vi "VIH - CHM Project - Create Project Files.vi"(8 "error in":errorcluster, 10 "HHP_Generation":T1={"HHP_Template"=enum."default", "HHP_Template_CustomPath"=path "", "HHP_Target"=enum."default", "HHP_Target_CustomPath"=path "", "HHP_CreateTOC"=TRUE, "HHP_CreateIDX"=TRUE, "HHP_DefaultTopic"=enum."auto", "HHP_DefaultTopic_CustomPath"=path "", "CHM_Filename"=path "", "HHP_AutoBuild"=FALSE, "CHM_AutoBuild"=FALSE}, 11 "Project Tree":T2) -> (0 "error out":errorcluster, 2 "Target HHP File":path, 3 "dup Project Tree":T2)   [LabVIEW 2014]
doc: "::: VI Helpeks :::\nCopyright (c) 2000-2026 Konstantin Shifershteyn. All rights reserved."
uses:
  _VIH Project Manager.llb/VIH Project Tree Typedef - Tree Refnum.ctl
  VIH - CHM Project - HHP Generation Params Cluster.ctl
panel:
  # "VI Helpeks\nCopyright (c) 2012-2026 Konstantin Shifershteyn"
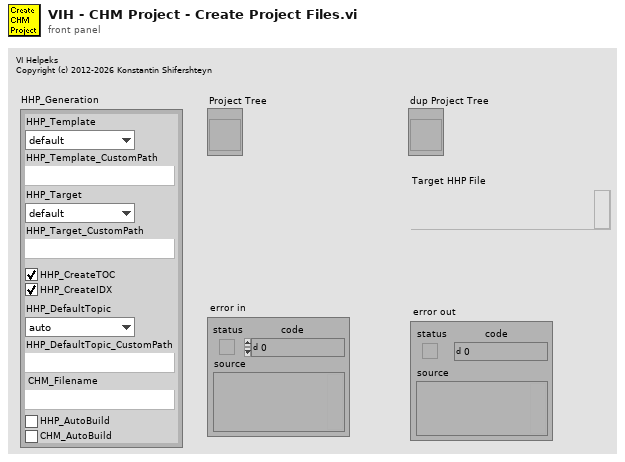
[diagram p1: front panel]
types:
  T1 = typedef "VIH - CHM Project - HHP Generation Params Cluster.ctl" = cluster{"HHP_Template":enum16{"default", "custom"}, "HHP_Template_CustomPath":path, "HHP_Target":enum16{"default", "custom"}, "HHP_Target_CustomPath":path, "HHP_CreateTOC":bool, "HHP_CreateIDX":bool, "HHP_DefaultTopic":enum16{"auto", "custom"}, "HHP_DefaultTopic_CustomPath":path, "CHM_Filename":path, "HHP_AutoBuild":bool, "CHM_AutoBuild":bool}
  T2 = typedef "VIH Project Tree Typedef - Tree Refnum.ctl" = refnum<vi>
  T3 = cluster{"TOC File":path, "IDX File":path, "HTML Files":path[], "Default Topic File":path, "Compiled File":path}
  T4 = typedef "VIH HelpGen Typedef - Palette - Item Type Enum.ctl" = enum32{"<Invalid>", "<unknown>", "VI", "Menu", "LV Func", "Express VI", "Poly VI", "CTL", "HTML"}
  T5 = cluster{"Types":T4[], "Src Paths":path[], "Dynamic":enum16{"Dyn", "Stat", "Both"}[], "HTML Paths":path[], "HTML Titles":string[]}
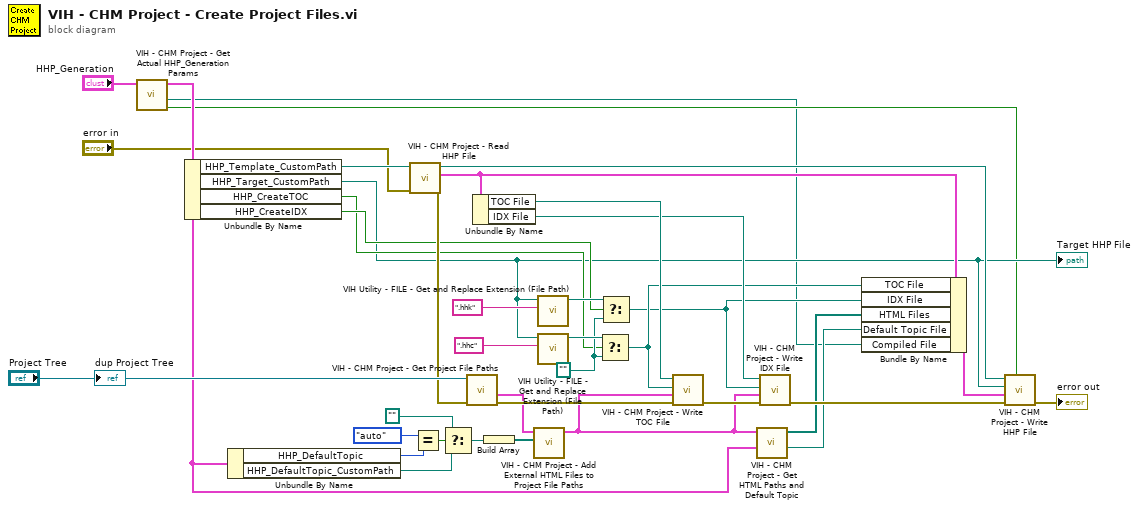
[diagram p0: block diagram]
diagram:
  w24 = path ""
  n1 = call "VIH - CHM Project - Get Actual HHP_Generation Params.vi"("HHP_Generation"="HHP_Generation") -> ("Abs CHM Path"=w4:bool, "CHM File Absolute Path"=w3:path, "HHP_Generation out"=w8:T1)  [unwired: 8 in]
  n2 = Unbundle By Name(w8) -> ("HHP_Template_CustomPath"=w36:path, "HHP_Target_CustomPath"=w7:path, "HHP_CreateTOC"=w19:bool, "HHP_CreateIDX"=w20:bool)
  "Target HHP File" <- w7
  n3 = Unbundle By Name(w8) -> ("HHP_DefaultTopic"=w16:enum16{"auto", "custom"}, "HHP_DefaultTopic_CustomPath"=w12:path)
  n4 = call "VIH - CHM Project - Read HHP File.vi"("error in"="error in", "HHP File"=w36) -> ("error out"=w29:errorcluster, "Files"=w23:T3, "dup HHP File"=w30:path)  [unwired: 7 in]
  n5 = Equal?(x=enum16{"auto", "custom"}."auto", y=w16) -> (x = y?=w15:bool)
  n6 = Select(t=path "", s=w15, f=w12) -> (s? t:f=w11:path)
  n7 = call "VIH - CHM Project - Get Project File Paths.vi"("error in"=w29, "Project Tree"="Project Tree") -> ("error out"=w35:errorcluster, "Project Files"=w18:T5)  [unwired: 7 in, 1 out]
  n8 = Unbundle By Name(w23) -> ("TOC File"=w28:path, "IDX File"=w27:path)
  n9 = Build Array(w11) -> (w17:path[])
  n10 = call "VIH - CHM Project - Add External HTML Files to Project File Paths.vi"("Extra HTML files"=w17, "Project Files"=w18) -> ("Project Files out"=w5:T5)  [unwired: 9 in]
  n11 = call "VIH Utility - FILE - Get and Replace Extension (File Path).vi"("new extension (none)"=".hhk", "file path"=w7) -> ("new file path"=w25:path)  [unwired: 8 in, 1 out]
  n12 = call "VIH Utility - FILE - Get and Replace Extension (File Path).vi"("new extension (none)"=".hhc", "file path"=w7) -> ("new file path"=w26:path)  [unwired: 8 in, 1 out]
  n13 = Select(t=w26, s=w19, f=w24) -> (s? t:f=w22:path)
  n14 = Select(t=w25, s=w20, f=w24) -> (s? t:f=w21:path)
  n15 = call "VIH - CHM Project - Write TOC File.vi"("error in"=w35, "Project Files"=w5, "Target TOC File"=w22, "Template TOC File"=w28) -> ("error out"=w33:errorcluster)  [unwired: 7 in]
  n16 = call "VIH - CHM Project - Get HTML Paths and Default Topic.vi"("HHP_Generation"=w8, "Project Files"=w5) -> ("Default Topic file"=w9:path, "HTML Files"=w10:path[])  [unwired: 8 in]
  n17 = call "VIH - CHM Project - Write IDX File.vi"("error in"=w33, "Project Files"=w5, "Target IDX File"=w21, "Template IDX File"=w27) -> ("error out"=w32:errorcluster)  [unwired: 7 in]
  n18 = Bundle By Name(cluster=w23, "TOC File"=w22, "IDX File"=w21, "HTML Files"=w10, "Default Topic File"=w9, "Compiled File"=w3) -> (w6:T3)
  n19 = call "VIH - CHM Project - Write HHP File.vi"("Abs CHM Path (F)"=w4, "error in"=w32, "Files"=w6, "Target HHP File"=w7, "Template HHP File"=w30) -> ("error out"=→"error out":errorcluster)  [unwired: 6 in]
  "dup Project Tree" <- "Project Tree"
